vi "PIDAutoTune_OpenLoopStep.vi"(7 "Configuration Parameters":T2={"Controller Constant Type"=enum."Ziegler Nicols - Normal", "Type of Controller"=enum."PI", "CO Offset"=0.25, "Kn"=1.0, "Tuning Tolerance"=0.001, "Plant Tolerance"=0.001, "Newest Avg Time "=1, "Long Ave Time"=6}, 8 "Sampling Time dt (s)":dbl=0.02, 9 "Tune":bool, 10 "Measurement  (PV)":dbl, 11 "Control Output (Co)":dbl) -> (0 "Plant and Test Data":T4, 1 "New Tuning Parameters":T3, 2 "Tuning Done":bool, 3 "Adj CO":dbl, 4 "Error Occured":bool, 6 "Diagnostic":T1)   [LabVIEW 2019, in "Trajectory_Library.lvlib"]
doc: "This routine can be used to make a step change to a PID control loop, track the results, and calculate PID tuning parameters. It wraps the NI LabVIEW PID auto-tuning functions for use with the WPILIB LabVIEW Math PID. This uses the OPEN LOOP STEP type of test. \n\nWarning -- This routine will modify the control output. Use it in such a manner to be able to stop the tuning if problems occur -- like running out of field space while tuning a drive motor. \n\nInputs:\n -- Configuration Parameters -- cluster -- This contains the parameters defining the conditions of the test. Use the Pack routine to create this data cluster.\n -- Control Output -- double -- The Control Output (CO) value from the output of the PID to be tuned.\n -- Measurement (PV) -- double -- The Process Variable (PV) value used by the PID to be tuned.\n -- Tune -- boolean -- When TRUE, tuning is performed..\n -- Sampling time -- double -- Loop time in seconds. How fast the PID and this autotune function are executed. (Optional: Default 0.02 seconds) \n\nOutputs:\n -- Adj CO -- double -- The adjusted CO. This is sent to the actuator. (This vi is put between the PID and the actuator device)\n -- Tuning Done -- boolean -- This is set to TRUE when tuning has completed. Depending on the PV noise, tuning may never be \"DONE\". However if the new tuning parameters are relatively constant, they can still be used.\n -- New Tuning Parameters -- cluster --- Data cluster containing the calculated PID tuning parameters. \n -- Plant and Test Data -- cluster -- Data cluster containing information describing the transfer function of the system being controlled (Plant).\n -- Error Occured -- Boolean -- If TRUE, an error occured.\n -- Diagnostic Info -- cluster -- This contains additional information about the test being perfromed."
uses:
  Trajectory_Library.lvlib
  Timer_New.vi
  LinearFilter_ResetToValue.vi
  LinearFilter_Calculate.vi
  <vilib>/Utility/semaphor.llb/Obtain Semaphore Reference.vi
  Timer_Reset.vi
  Timer_Start.vi
  Timer_Stop.vi
  Timer_HasPeriodPassedOnce.vi
  <vilib>/addons/control/pid/autopid.llb/PID Autotuning Design (Auto).vi
  <vilib>/addons/control/pid/autopid.llb/PID Autotuning Design (Chien-Hrones-Reswick).vi
  LinearFilter_MovingAverage.vi
  LinearFilter_LowPassBW1.vi
  LinearFilter_LowPassBW2.vi
  LinearFilter_HighPassBW1.vi
  LinearFilter_HighPassBW2.vi
  <vilib>/Analysis/Matrix/Numeric/Conversions/Array To Matrix - RA.vi
  <vilib>/addons/control/pid/NI_PID_autopid.lvlib
  <vilib>/ptbypt/NI_PtbyPt.lvlib
  <vilib>/Analysis/Matrix/NI_Matrix.lvlib
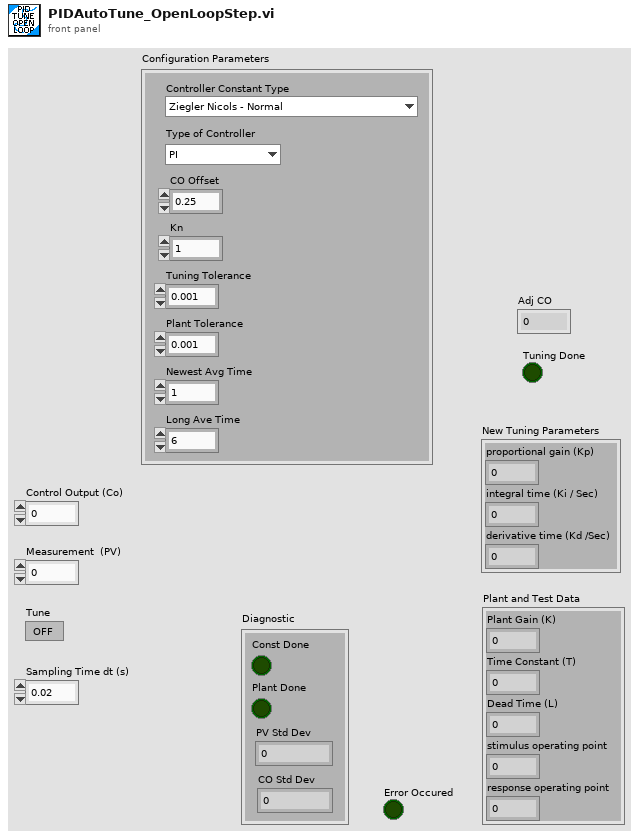
[diagram p1: front panel]
types:
  T1 = cluster{"Const Done":bool, "Plant Done":bool, "PV Std Dev":dbl, "CO Std Dev":dbl}
  T2 = cluster{"Controller Constant Type":enum16{"Ziegler Nicols - Fast", "Ziegler Nicols - Normal", "Ziegler Nicols - Slow", "CHR regulator - 0% overshoot", "CHR regulator - 20% overshoot", "CHR servo - 0 % overshoot", "CHR servo - 20% overshoot"}, "Type of Controller":enum16{"P", "PI", "PID"}, "CO Offset":dbl, "Kn":dbl, "Tuning Tolerance":dbl, "Plant Tolerance":dbl, "Newest Avg Time ":i32, "Long Ave Time":i32}
  T3 = cluster{"proportional gain (Kp)":dbl, "integral time (Ki / Sec)":dbl, "derivative time (Kd /Sec)":dbl}
  T4 = cluster{"Plant Gain (K)":dbl, "Time Constant (T)":dbl, "Dead Time (L)":dbl, "stimulus operating point":dbl, "response operating point":dbl}
  T5 = enum16{"Ziegler Nicols - Fast", "Ziegler Nicols - Normal", "Ziegler Nicols - Slow", "CHR regulator - 0% overshoot", "CHR regulator - 20% overshoot", "CHR servo - 0 % overshoot", "CHR servo - 20% overshoot"}
  T6 = cluster{"proportional gain (Kc)":dbl, "integral time (Ti, min)":dbl, "derivative time (Td, min)":dbl}
  T7 = cluster{"Plant Gain (K)":dbl, "Time Constant (T)":dbl, "Dead Time (L)":dbl}
  T8 = cluster{"Plant Gain (K)":dbl, "Time Constant (T)":dbl, "Dead Time (L)":dbl, "stimulus offset":dbl, "response offset":dbl}
  T9 = typedef "NI_Matrix.lvlib/RealMatrix.ctl" = dbl[][]
  T10 = cluster{"WithinTolerance":bool, "WithinTolerance":bool, "standard deviation":dbl, "standard deviation":dbl}
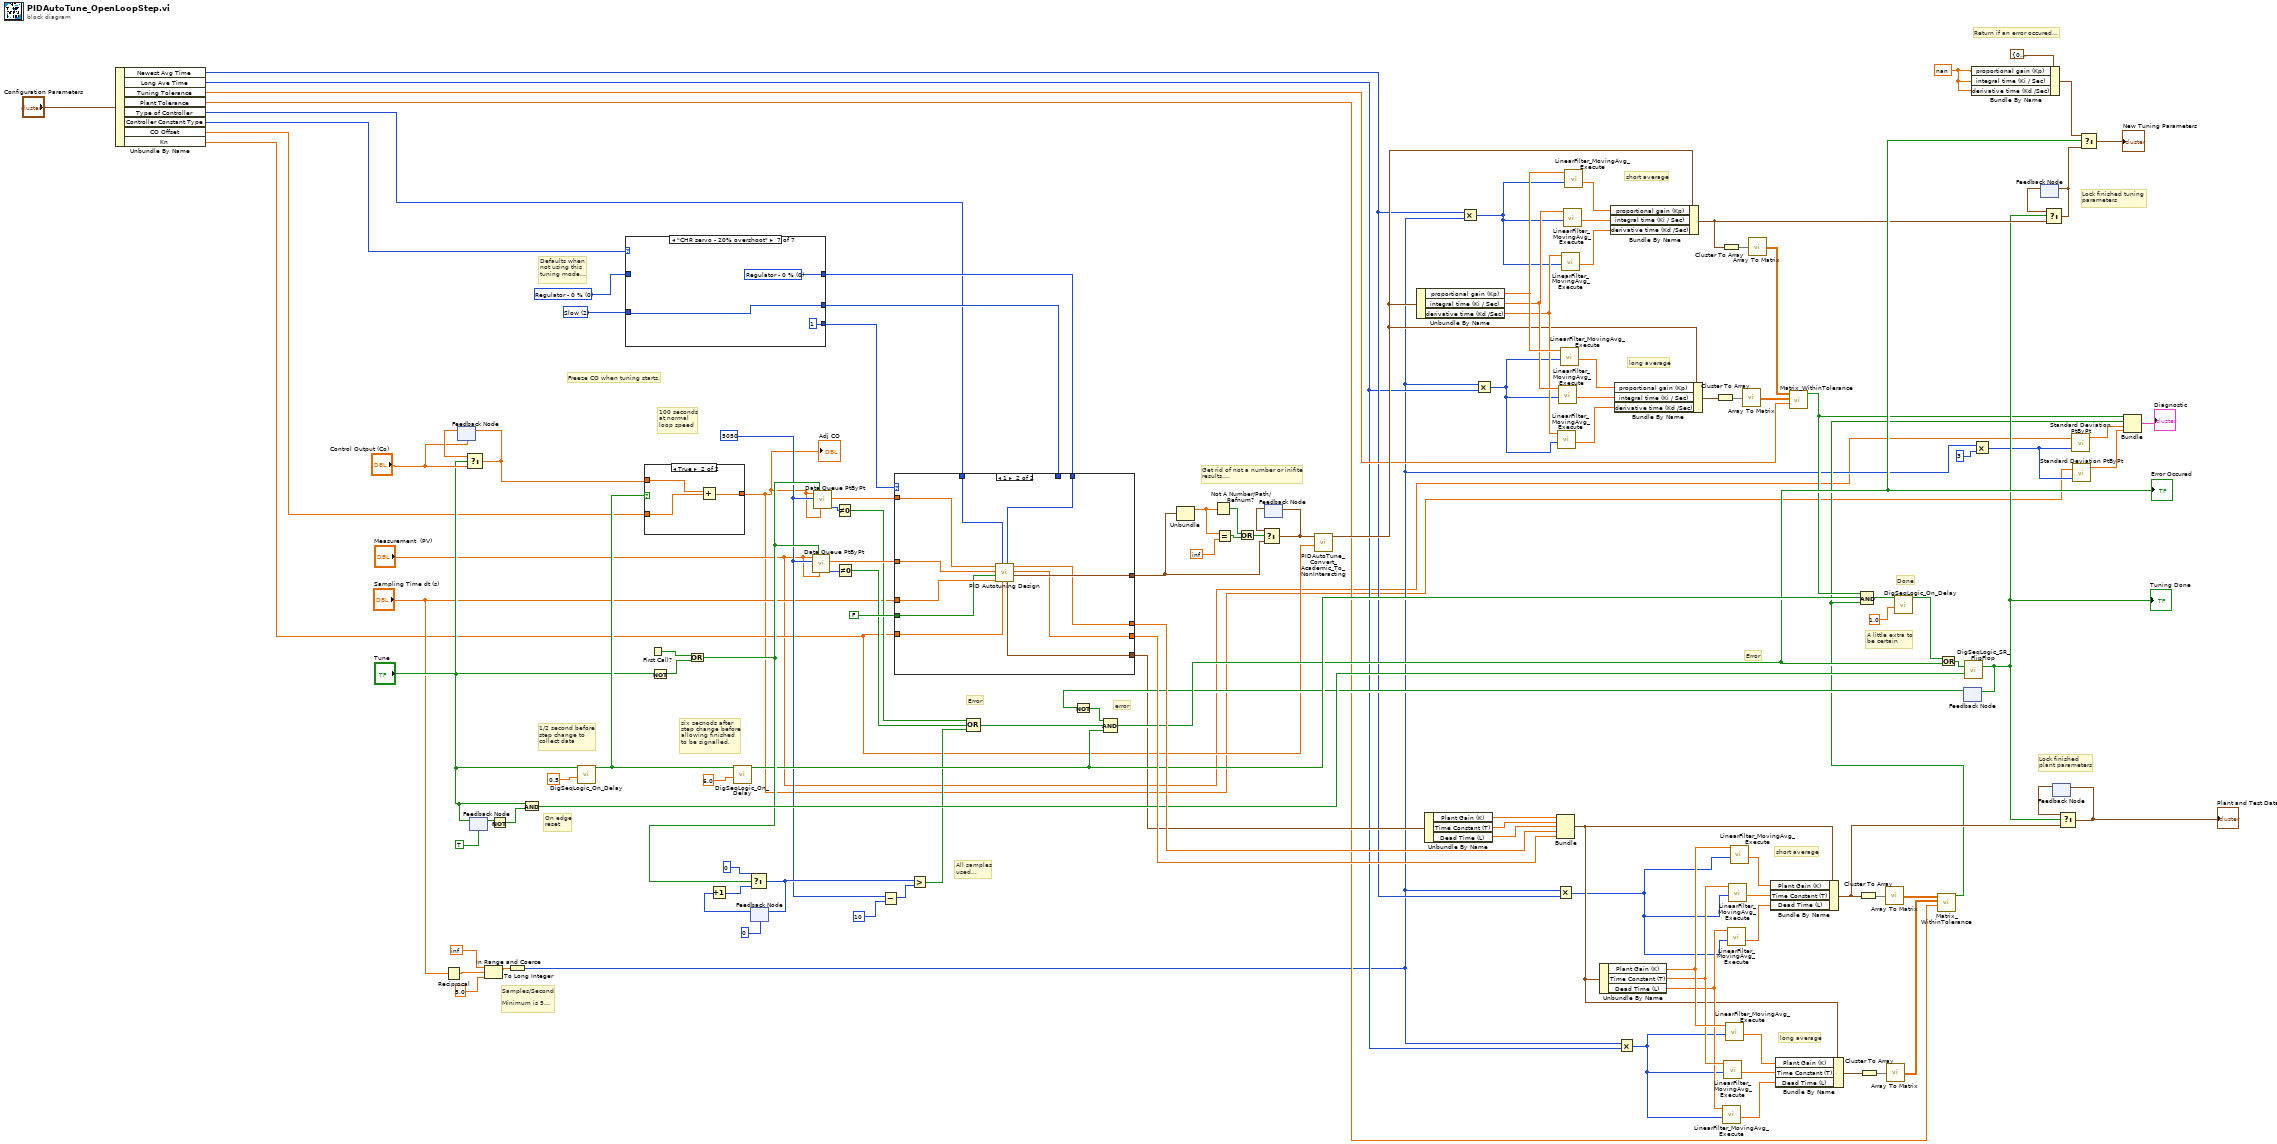
[diagram p0: block diagram]
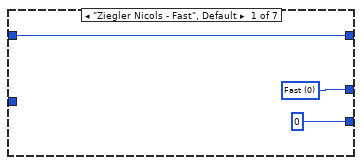
[diagram p2: hidden frame]
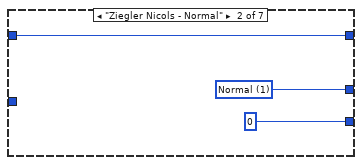
[diagram p3: hidden frame]
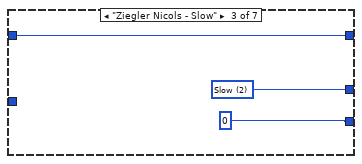
[diagram p4: hidden frame]
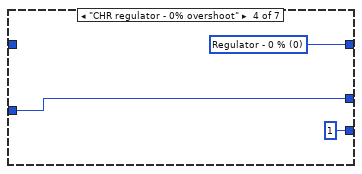
[diagram p5: hidden frame]
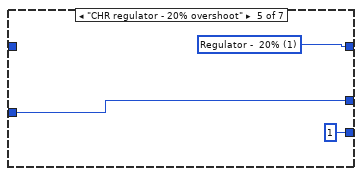
[diagram p6: hidden frame]
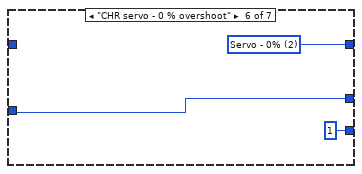
[diagram p7: hidden frame]
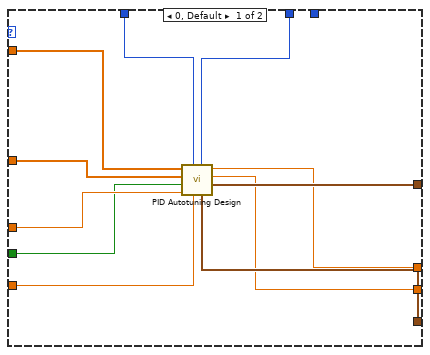
[diagram p8: hidden frame]
diagram:
  w81 = nan
  w96 = u16 2 items=["Fast", "Normal", "Slow"] ("Ziegler-Nichols Speed")
  w97 = u16 0 items=["Regulator - 0 %", "Regulator -  20%", "Servo - 0%", "Servo - 20%"] ("Tuning specifications")
  w68 = 5050 ("sample length")
  # "Get rid of not a number or inifite\nresults...."
  # "On edge\nreset"
  # "Error"
  # "All samples\nused..."
  # "Error"
  # "Done"
  # "Lock finished \nplant parameters"
  # "Lock finished tuning\nparameters"
  # "Samples/Second\n\nMinimum is 5..."
  # "long average"
  # "short average"
  # "long average"
  # "short average"
  # "error"
  # "Return if an error occured..."
  # "A little extra to\nbe certain"
  # "Defaults when\nnot using this\ntuning mode..."
  # "100 seconds\nat normal\nloop speed"
  # "Freeze CO when tuning starts."
  # "six secnods after\nstep change before\nallowing finished \nto be signalled."
  # "1/2 second before\nstep change to\ncollect data"
  n1 = Unbundle By Name("Configuration Parameters") -> ("Newest Avg Time"=w12:i32, "Long Ave Time"=w11:i32, "Tuning Tolerance"=w17:dbl, "Plant Tolerance"=w16:dbl, "Type of Controller"=w20:enum16{"P", "PI", "PID"}, "Controller Constant Type"=w21:T5, "CO Offset"=w19:dbl, "Kn"=w18:dbl)
  n2 = Reciprocal(x="Sampling Time dt (s)") -> (1/x=w58:dbl)
  n3 = feedback #1("Control Output (Co)") -> (w112:dbl)
  n4 = Select(t=w112, s="Tune", f="Control Output (Co)") -> (s? t:f=w113:dbl)
  n5 = feedback-in #1(w113) -> ()
  n6 = feedback-in #2("Tune") -> ()
  n7 = feedback #2(TRUE ("Tune")) -> (w109:bool)
  n8 = In Range and Coerce(upper limit=inf, x=w58, lower limit=5.0) -> (coerced(x)=w49:dbl)  [unwired: 1 out]
  n9 = Not(x=w109) -> (.not. x?=w107:bool)
  n10 = To Long Integer(number=w49) -> (32bit integer=w6:i32)
  n11 = And(x="Tune", y=w107) -> (x .and. y?=w106:bool)
  n12 = call "DigSeqLogic_On_Delay.vi"("Delay"=0.5, "Input"="Tune") -> ("Output"=w114:bool)  [unwired: 8 in, 1 out]
  n13 = case shown="\"CHR servo - 20% overshoot\"" w21 {
    tunnel: [w130 w133 w136 w137 w140 w143 w146] -> w100
    tunnel: [0 0 0 1 1 1 1] -> w99
    tunnel: [w128 w131 w134 w138 w141 w144 w147] -> w98
    tunnel: w97 -> [w128 w131 w134 _ _ _ _]
    tunnel: w96 -> [_ _ _ w137 w140 w143 w146]
    frame "Ziegler Nicols - Fast", Default {
      w130 = u16 0 items=["Fast", "Normal", "Slow"] ("Ziegler-Nichols Speed")
    }
    frame "Ziegler Nicols - Normal" {
      w133 = u16 1 items=["Fast", "Normal", "Slow"] ("Ziegler-Nichols Speed")
    }
    frame "Ziegler Nicols - Slow" {
      w136 = u16 2 items=["Fast", "Normal", "Slow"] ("Ziegler-Nichols Speed")
    }
    frame "CHR regulator - 0% overshoot" {
      w138 = u16 0 items=["Regulator - 0 %", "Regulator -  20%", "Servo - 0%", "Servo - 20%"] ("Tuning specifications")
    }
    frame "CHR regulator - 20% overshoot" {
      w141 = u16 1 items=["Regulator - 0 %", "Regulator -  20%", "Servo - 0%", "Servo - 20%"] ("Tuning specifications")
    }
    frame "CHR servo - 0 % overshoot" {
      w144 = u16 2 items=["Regulator - 0 %", "Regulator -  20%", "Servo - 0%", "Servo - 20%"] ("Tuning specifications")
    }
    frame "CHR servo - 20% overshoot" {
      w147 = u16 0 items=["Regulator - 0 %", "Regulator -  20%", "Servo - 0%", "Servo - 20%"] ("Tuning specifications")
    }
  }
  n14 = case shown="True" w114 {
    tunnel: w113 -> [w149 w152]
    tunnel: w19 -> [_ w151]
    tunnel: [w149 w150] -> w2
    frame False {
    }
    frame True {
      n15 = Add(x=w152, y=w151) -> (x+y=w150:dbl)
    }
  }
  "Adj CO" <- w2
  n16 = First Call?() -> (First Call?: T/F=w80:bool)
  n17 = Not(x="Tune") -> (.not. x?=w79:bool)
  n18 = Or(x=w80, y=w79) -> (x .or. y?=w77:bool)
  n19 = call "DigSeqLogic_On_Delay.vi"("Delay"=6.0, "Input"=w114) -> ("Output"=w75:bool)  [unwired: 8 in, 1 out]
  n20 = feedback #3(0) -> (w72:i32)
  n21 = Increment(x=w72) -> (x+1=w71:i32)
  n22 = Select(t=0, s=w77, f=w71) -> (s? t:f=w70:i32)
  n23 = feedback-in #3(w70) -> ()
  n24 = call <vilib>:"Data Queue PtByPt.vi"("initial queue element"="Measurement  (PV)", "initialize"=w77, "sample length"=w68, "input data point"="Measurement  (PV)") -> ("error"=w88:i32, "Current Queue"=w122:dbl[])  [unwired: 3 in, 3 out]
  n25 = call <vilib>:"Data Queue PtByPt.vi"("initial queue element"=w2, "initialize"=w77, "sample length"=w68, "input data point"=w2) -> ("error"=w89:i32, "Current Queue"=w123:dbl[])  [unwired: 3 in, 3 out]
  n26 = Not Equal To 0?(x=w89) -> (x != 0?=w65:bool)
  n27 = Not Equal To 0?(x=w88) -> (x != 0?=w64:bool)
  n28 = Subtract(x=w68, y=10) -> (x-y=w69:i32)
  n29 = case shown="1" w99 {
    tunnel: [w163 w174] -> w126
    tunnel: "Sampling Time dt (s)" -> [w162 w173]
    tunnel: w123 -> [w161 w172]
    tunnel: w122 -> [w160 w171]
    tunnel: w20 -> [w159 w170]
    tunnel: [w158 w169] -> w30
    tunnel: [w157 w168] -> w118
    tunnel: [w156 w167] -> w117
    tunnel: w18 -> [w155 w166]
    tunnel: w100 -> [w154 _]
    tunnel: w98 -> [_ w165]
    tunnel: FALSE ("closed-loop?") -> [w153 w164]
    frame 0, Default {
      n30 = call-poly <vilib>:"PID Autotuning Design.vi"("Ziegler-Nichols Speed"=w154, "Controller Gain (K)"=w155, "Type of Controller"=w159, "dt (s)"=w162, "closed-loop?"=w153, "Response signal"=w160, "Stimulus signal"=w161) -> ("PID gains"=w163:T6, "response operating point"=w156:dbl, "stimulus operating point"=w157:dbl, "Plant Parameters"=w158:T7)  [unwired: 1 in]
    }
    frame 1 {
      n31 = call-poly <vilib>:"PID Autotuning Design.vi"("Tuning specifications"=w165, "Controller Gain (K)"=w166, "Type of Controller"=w170, "dt (s)"=w173, "closed-loop?"=w164, "Response signal"=w171, "Stimulus signal"=w172) -> ("PID gains"=w174:T6, "response offset"=w167:dbl, "stimulus offset"=w168:dbl, "Plant Parameters"=w169:T7)  [unwired: 1 in]
    }
  }
  n32 = Greater?(x=w70, y=w69) -> (0:w66:bool)
  n33 = Compound Arithmetic op=OR(w65, w64, w66) -> (w76:bool)
  n34 = Unbundle(w126) -> ("proportional gain (Kc)"=w61:dbl)  [unwired: 2 out]
  n35 = Not A Number/Path/Refnum?(number/path/refnum=w61) -> (NaN/Path/Refnum?=w60:bool)
  n36 = Equal?(x=w61, y=inf) -> (x = y?=w90:bool)
  n37 = Or(x=w60, y=w90) -> (x .or. y?=w91:bool)
  n38 = feedback #4() -> (w125:T6)  [unwired: 1 in]
  n39 = Select(t=w125, s=w91, f=w126) -> (s? t:f=w127:T6)
  n40 = feedback-in #4(w127) -> ()
  n41 = call "PIDAutoTune_Convert_Academic_To_NonInteracting.vi"("Kn"=w18, "PID gains NI Academic"=w127) -> ("PID Gains Non Interacting"=w45:T3)  [unwired: 9 in]
  n42 = Unbundle By Name(w45) -> ("proportional gain (Kp)"=w52:dbl, "integral time (Ki / Sec)"=w51:dbl, "derivative time (Kd /Sec)"=w50:dbl)
  n43 = Unbundle By Name(w30) -> ("Plant Gain (K)"=w121:dbl, "Time Constant (T)"=w120:dbl, "Dead Time (L)"=w119:dbl)
  n44 = Multiply(x=w12, y=w6) -> (x*y=w15:i32)
  n45 = Multiply(x=w6, y=w11) -> (x*y=w48:i32)
  n46 = Bundle("Plant Gain (K)"=w121, "Time Constant (T)"=w120, "Dead Time (L)"=w119, "stimulus offset"=w118, "response offset"=w117) -> (w29:T8)  [unwired: 1 in]
  n47 = Multiply(x=w6, y=w12) -> (x*y=w13:i32)
  n48 = call "LinearFilter_MovingAvg_Execute.vi"("Samples"=w48, "Input"=w50) -> ("Output"=w53:dbl)  [unwired: 9 in]
  n49 = call "LinearFilter_MovingAvg_Execute.vi"("Samples"=w48, "Input"=w51) -> ("Output"=w55:dbl)  [unwired: 9 in]
  n50 = call "LinearFilter_MovingAvg_Execute.vi"("Samples"=w48, "Input"=w52) -> ("Output"=w54:dbl)  [unwired: 9 in]
  n51 = call "LinearFilter_MovingAvg_Execute.vi"("Samples"=w15, "Input"=w50) -> ("Output"=w92:dbl)  [unwired: 9 in]
  n52 = call "LinearFilter_MovingAvg_Execute.vi"("Samples"=w15, "Input"=w51) -> ("Output"=w93:dbl)  [unwired: 9 in]
  n53 = call "LinearFilter_MovingAvg_Execute.vi"("Samples"=w15, "Input"=w52) -> ("Output"=w94:dbl)  [unwired: 9 in]
  n54 = Unbundle By Name(w29) -> ("Plant Gain (K)"=w34:dbl, "Time Constant (T)"=w33:dbl, "Dead Time (L)"=w32:dbl)
  n55 = Bundle By Name(cluster=w45, "proportional gain (Kp)"=w94, "integral time (Ki / Sec)"=w93, "derivative time (Kd /Sec)"=w92) -> (w44:T3)
  n56 = Bundle By Name(cluster=w45, "proportional gain (Kp)"=w54, "integral time (Ki / Sec)"=w55, "derivative time (Kd /Sec)"=w53) -> (w47:T3)
  n57 = Multiply(x=w6, y=w11) -> (x*y=w31:i32)
  n58 = Cluster To Array(cluster=w47) -> (array=w46:dbl[])
  n59 = Cluster To Array(cluster=w44) -> (array=w43:dbl[])
  n60 = call "LinearFilter_MovingAvg_Execute.vi"("Samples"=w31, "Input"=w32) -> ("Output"=w35:dbl)  [unwired: 9 in]
  n61 = call "LinearFilter_MovingAvg_Execute.vi"("Samples"=w31, "Input"=w33) -> ("Output"=w37:dbl)  [unwired: 9 in]
  n62 = call "LinearFilter_MovingAvg_Execute.vi"("Samples"=w31, "Input"=w34) -> ("Output"=w36:dbl)  [unwired: 9 in]
  n63 = call "LinearFilter_MovingAvg_Execute.vi"("Samples"=w13, "Input"=w32) -> ("Output"=w38:dbl)  [unwired: 9 in]
  n64 = call "LinearFilter_MovingAvg_Execute.vi"("Samples"=w13, "Input"=w33) -> ("Output"=w39:dbl)  [unwired: 9 in]
  n65 = call "LinearFilter_MovingAvg_Execute.vi"("Samples"=w13, "Input"=w34) -> ("Output"=w40:dbl)  [unwired: 9 in]
  n66 = call-poly <vilib>:"Array To Matrix.vi"("Real 1D Array"=w46) -> ("Real Matrix (Column Vector)"=w42:T9)
  n67 = call-poly <vilib>:"Array To Matrix.vi"("Real 1D Array"=w43) -> ("Real Matrix (Column Vector)"=w41:T9)
  n68 = Bundle By Name(cluster=w29, "Plant Gain (K)"=w40, "Time Constant (T)"=w39, "Dead Time (L)"=w38) -> (w25:T8)
  n69 = Bundle By Name(cluster=w29, "Plant Gain (K)"=w36, "Time Constant (T)"=w37, "Dead Time (L)"=w35) -> (w26:T8)
  n70 = call "Matrix_WithinTolerance.vi"("Tolerance"=w17, "Matrix B"=w42, "Matrix A"=w41) -> ("WithinTolerance"=w9:bool)  [unwired: 7 in, 1 out]
  n71 = Cluster To Array(cluster=w25) -> (array=w28:dbl[])
  n72 = Cluster To Array(cluster=w26) -> (array=w27:dbl[])
  n73 = call-poly <vilib>:"Array To Matrix.vi"("Real 1D Array"=w28) -> ("Real Matrix (Column Vector)"=w24:T9)
  n74 = call-poly <vilib>:"Array To Matrix.vi"("Real 1D Array"=w27) -> ("Real Matrix (Column Vector)"=w23:T9)
  n75 = call "Matrix_WithinTolerance.vi"("Tolerance"=w16, "Matrix B"=w23, "Matrix A"=w24) -> ("WithinTolerance"=w8:bool)  [unwired: 7 in, 1 out]
  n76 = Compound Arithmetic op=AND(w9, w75, w8) -> (w102:bool)
  n77 = call "DigSeqLogic_On_Delay.vi"("Delay"=1.0, "Input"=w102) -> ("Output"=w86:bool)  [unwired: 8 in, 1 out]
  n78 = feedback #5() -> (w62:bool)  [unwired: 1 in]
  n79 = Not(x=w62) -> (.not. x?=w63:bool)
  n80 = Compound Arithmetic op=AND(w63, w76, w75) -> (w74:bool)
  "Error Occured" <- w74
  n81 = Or(x=w86, y=w74) -> (x .or. y?=w87:bool)
  n82 = call "DigSeqLogic_SR_FlipFlop.vi"("Set"=w87, "Reset"=w106) -> ("Output"=w14:bool)  [unwired: 12 in, 1 out]
  "Tuning Done" <- w14
  n83 = feedback-in #5(w14) -> ()
  n84 = Bundle By Name(cluster=T3 {"proportional gain (Kp)"=0.0, "integral time (Ki / Sec)"=0.0, "derivative time (Kd /Sec)"=0.0} ("t"), "proportional gain (Kp)"=w81, "integral time (Ki / Sec)"=w81, "derivative time (Kd /Sec)"=w81) -> (w82:T3)
  n85 = Multiply(x=w6, y=3) -> (x*y=w3:i32)
  n86 = feedback #6() -> (w103:T3)  [unwired: 1 in]
  n87 = Select(t=w103, s=w14, f=w44) -> (s? t:f=w84:T3)
  n88 = feedback-in #6(w84) -> ()
  n89 = feedback #7() -> (w104:T8)  [unwired: 1 in]
  n90 = Select(t=w104, s=w14, f=w25) -> (s? t:f=w105:T8)
  "Plant and Test Data" <- w105
  n91 = feedback-in #7(w105) -> ()
  n92 = call <vilib>:"Standard Deviation PtByPt.vi"("x"="Measurement  (PV)", "sample length"=w3) -> ("standard deviation"=w7:dbl)  [unwired: 1 in, 2 out]
  n93 = call <vilib>:"Standard Deviation PtByPt.vi"("x"=w2, "sample length"=w3) -> ("standard deviation"=w1:dbl)  [unwired: 1 in, 2 out]
  n94 = Select(t=w82, s=w74, f=w84) -> (s? t:f=→"New Tuning Parameters":T3)
  n95 = Bundle("WithinTolerance"=w9, "WithinTolerance"=w8, "standard deviation"=w7, "standard deviation"=w1) -> (→"Diagnostic":T10)  [unwired: 1 in]
